vi "Get Report String.vi"(8 "error in (no error)":errorcluster, 11 "TestStand Result Handler In":refnum<class "TestStand Result Handler.lvclass">) -> (0 "error out":errorcluster, 2 "Report Text":string)   [LabVIEW 2020, in "Astemes_CSVReportPlugin.lvlib" / "TestStand Result Handler.lvclass"]
uses:
  TestStand Result Handler.lvclass
  TestStand Result Handler.lvclass/TestStand Result Handler.ctl
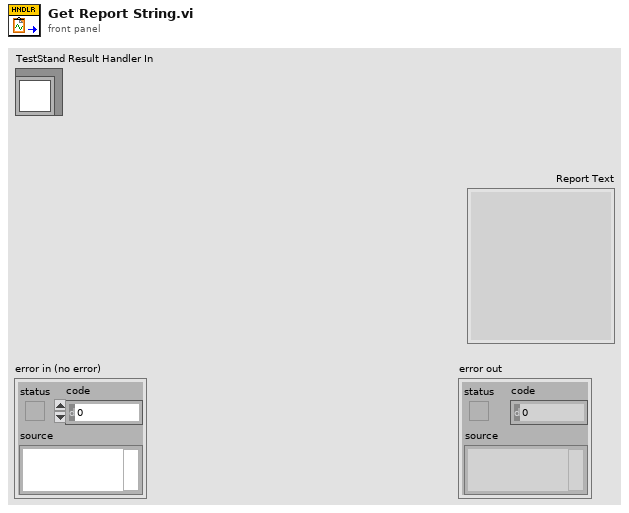
[diagram p1: front panel]
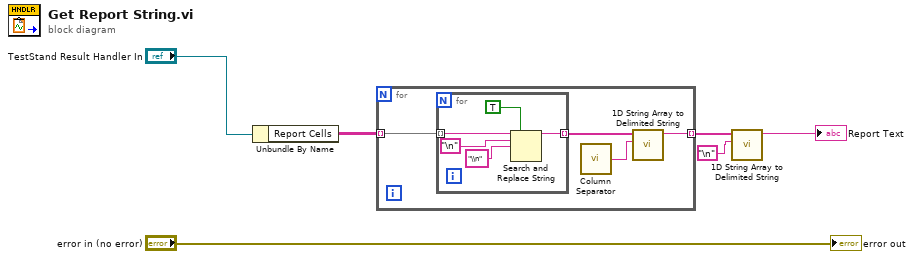
[diagram p0: block diagram]
diagram:
  n1 = Unbundle By Name("TestStand Result Handler In") -> ("Report Cells"=w4:string[][])
  n2 = for {
    tunnel: w4 -> [w7] mode=indexing
    tunnel: [w10] -> w3 mode=indexing
    n3 = for {
      tunnel: [w11] -> w8 mode=indexing
      tunnel: w7 -> [w12] mode=indexing
      n4 = Search and Replace String(replace all?=TRUE ("replace all? (F)"), input string=w12, search string="\n", replace string="\\n") -> (result string=w11:string)  [unwired: 4 in, 3 out]
    }
    n5 = call "Column Separator.vi"() -> ("delimiter"=w9:string)
    n6 = call <vilib>:"1D String Array to Delimited String.vi"("delimiter"=w9, "string array"=w8) -> ("delimited string"=w10:string)  [unwired: 9 in]
  }
  n7 = call <vilib>:"1D String Array to Delimited String.vi"("delimiter"="\n", "string array"=w3) -> ("delimited string"=→"Report Text":string)  [unwired: 9 in]
  "error out" <- "error in (no error)"
